vi "Game_Undo_Move.vi"(0 "Context":T1={"Screen"=enum."Settings", "Settings"=[0, 0, 1, 1], "Board"={"Grid"=array15x15[225 elements], "Move History"=[], "Last Move"={"Row"=-1, "Col"=-1, "Stone"=enum."Empty"}}, "Status"=enum."Idle", "Game ID"=0, "Player Stone"=enum."Black", "Hover"={"Row"=-1, "Col"=-1, "Stone"=enum."Empty"}, "Hover Button"=-1, "Win Line"=[], "Score 1"=0, "Score 2"=0, "Draws"=0, "Status Text"="", "Status Color"=0}, 11 "error in":errorcluster) -> (4 "Context out":T1={"Screen"=enum."Settings", "Settings"=[0, 0, 1, 1], "Board"={"Grid"=array15x15[225 elements], "Move History"=[], "Last Move"={"Row"=-1, "Col"=-1, "Stone"=enum."Empty"}}, "Status"=enum."Idle", "Game ID"=0, "Player Stone"=enum."Black", "Hover"={"Row"=-1, "Col"=-1, "Stone"=enum."Empty"}, "Hover Button"=-1, "Win Line"=[], "Score 1"=0, "Score 2"=0, "Draws"=0, "Status Text"="", "Status Color"=0}, 15 "error out":errorcluster)   [LabVIEW 2026]
doc: "무르기 버튼: 2인 플레이는 1수, AI 대전은 플레이어 차례가 되도록 1~2수(AI 흑 첫 수는 유지).\nGame ID를 올려 계산 중이던 AI 결과를 버린다."
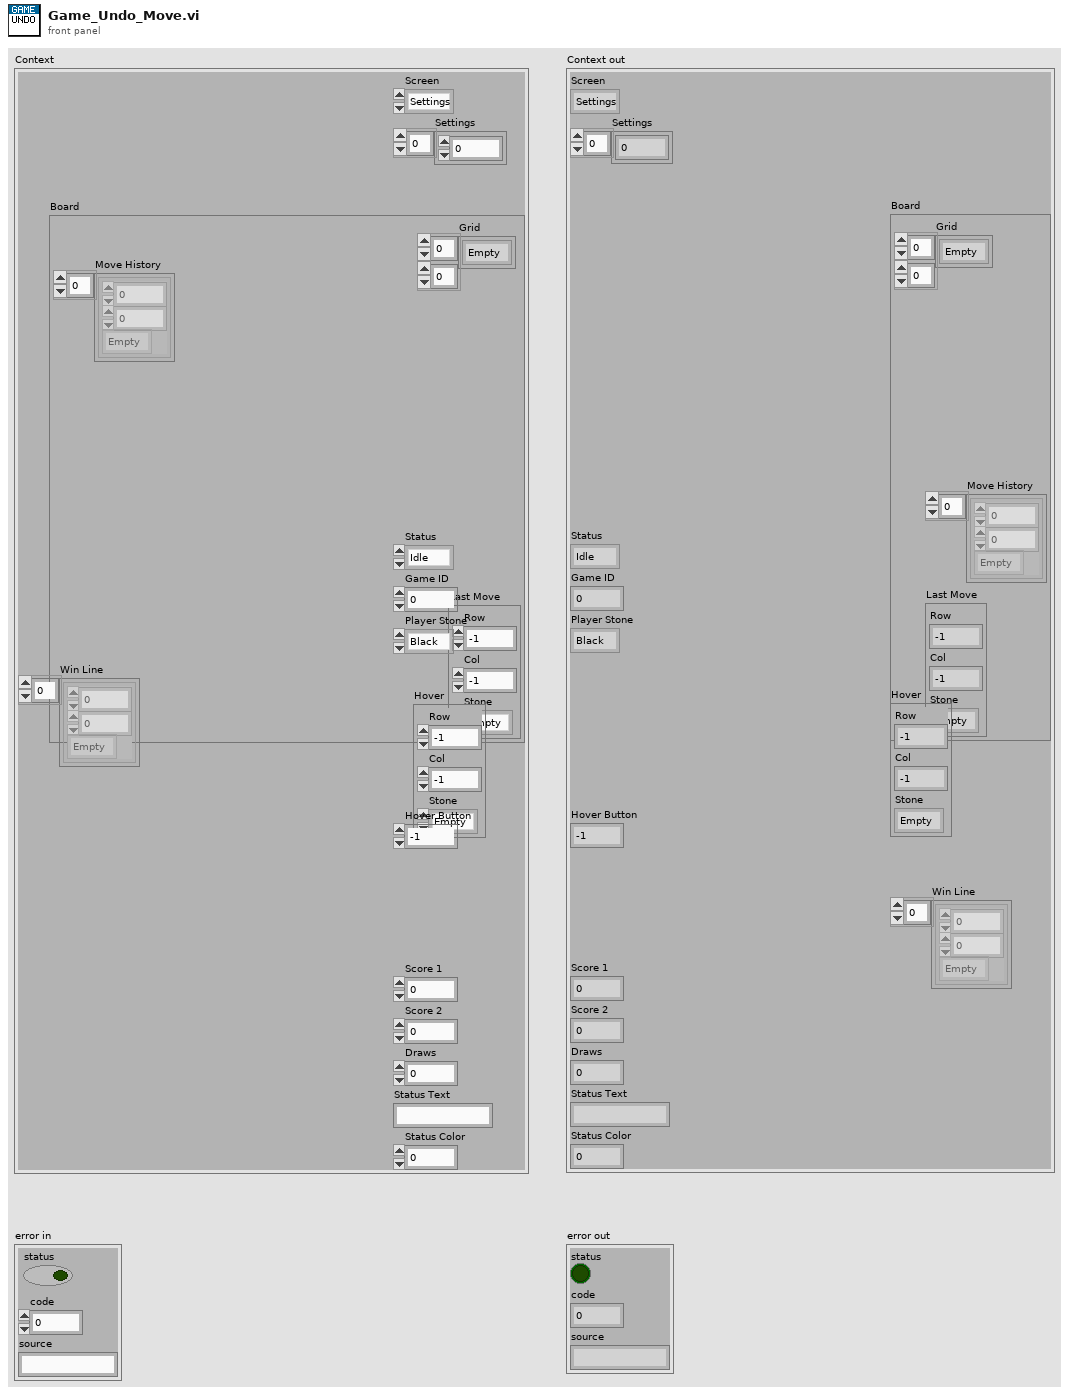
[diagram p1: front panel]
types:
  T1 = cluster{"Screen":enum16{"Settings", "Game"}, "Settings":i32[], "Board":cluster{"Grid":enum8{"Empty", "Black", "White"}[][], "Move History":cluster{"Row":i32, "Col":i32, "Stone":enum8{"Empty", "Black", "White"}}[], "Last Move":cluster{"Row":i32, "Col":i32, "Stone":enum8{"Empty", "Black", "White"}}}, "Status":enum16{"Idle", "Player Turn", "AI Thinking", "Game Over"}, "Game ID":u32, "Player Stone":enum8{"Empty", "Black", "White"}, "Hover":cluster{"Row":i32, "Col":i32, "Stone":enum8{"Empty", "Black", "White"}}, "Hover Button":i32, "Win Line":cluster{"Row":i32, "Col":i32, "Stone":enum8{"Empty", "Black", "White"}}[], "Score 1":i32, "Score 2":i32, "Draws":i32, "Status Text":string, "Status Color":u32}
  T2 = enum16{"Idle", "Player Turn", "AI Thinking", "Game Over"}
  T3 = cluster{"Row":i32, "Col":i32, "Stone":enum8{"Empty", "Black", "White"}}[]
  T4 = cluster{"Grid":enum8{"Empty", "Black", "White"}[][], "Move History":cluster{"Row":i32, "Col":i32, "Stone":enum8{"Empty", "Black", "White"}}[], "Last Move":cluster{"Row":i32, "Col":i32, "Stone":enum8{"Empty", "Black", "White"}}}
  T5 = cluster{"Row":i32, "Col":i32, "Stone":enum8{"Empty", "Black", "White"}}
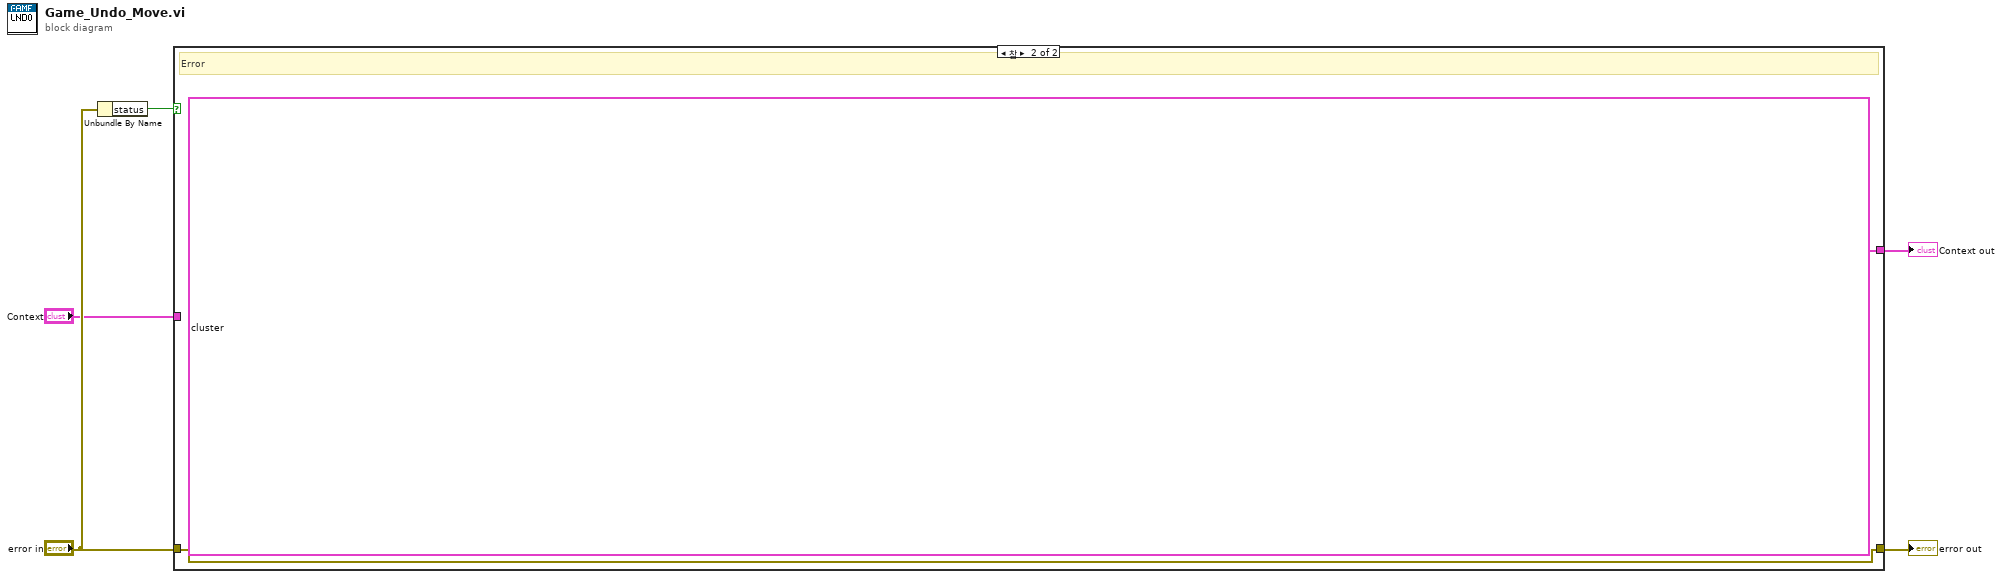
[diagram p0: block diagram]
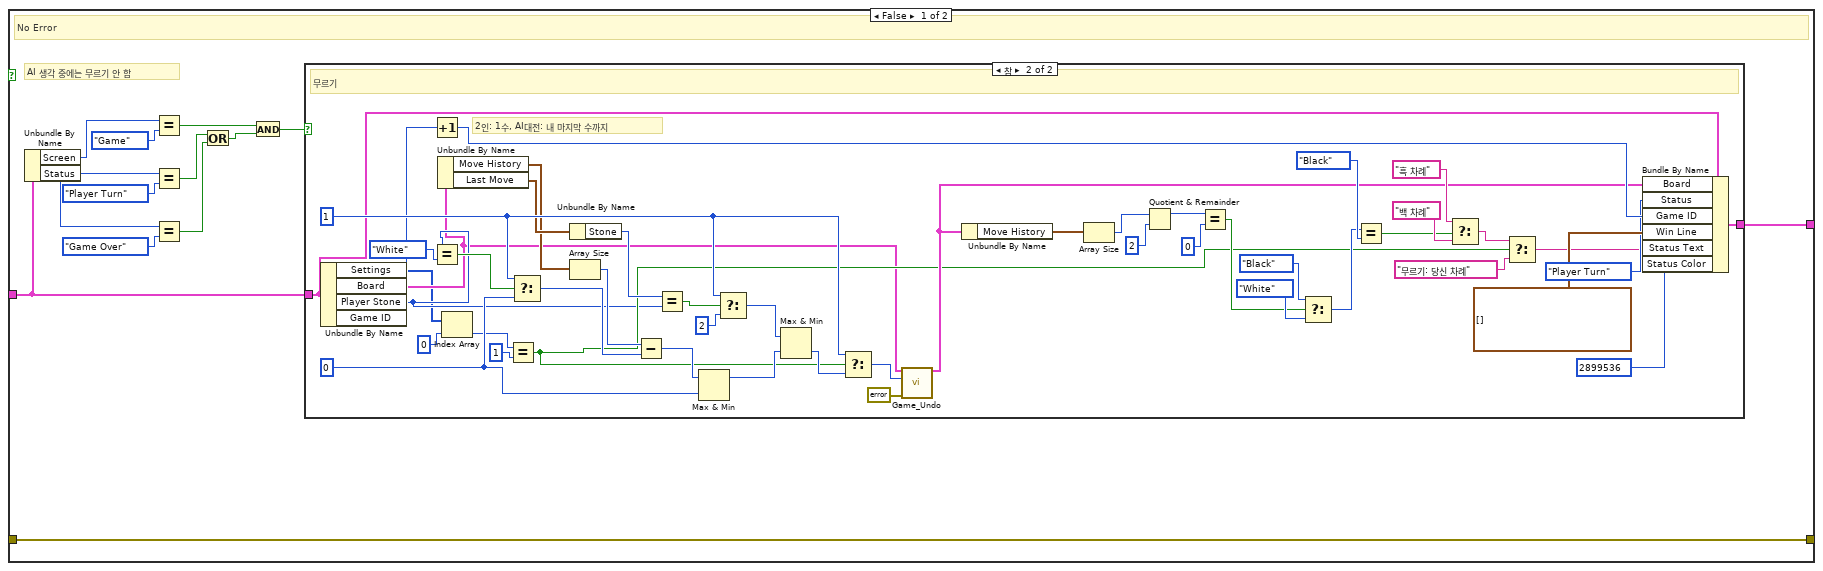
[diagram p2: hidden frame]
diagram:
  n1 = Unbundle By Name("error in") -> ("status"=w3:bool)
  n2 = case shown="참" w3 {
    tunnel: "Context" -> [w6 _]
    tunnel: "error in" -> [w7 w68]
    tunnel: [w7 w68] -> w5
    tunnel: [w18 T1 {"Screen"=enum."Settings", "Settings"=[0, 0, 1, 1], "Board"={"Grid"=array15x15[225 elements], "Move History"=[], "Last Move"={"Row"=-1, "Col"=-1, "Stone"=enum."Empty"}}, "Status"=enum."Idle", "Game ID"=0, "Player Stone"=enum."Black", "Hover"={"Row"=-1, "Col"=-1, "Stone"=enum."Empty"}, "Hover Button"=-1, "Win Line"=[], "Score 1"=0, "Score 2"=0, "Draws"=0, "Status Text"="", "Status Color"=0}] -> w4
    frame False {
      # "AI 생각 중에는 무르기 안 함"
      # "No Error"
      n3 = Unbundle By Name(w6) -> ("Screen"=w8:enum16{"Settings", "Game"}, "Status"=w9:T2)
      n4 = Equal?(x=w8, y=enum16{"Settings", "Game"}."Game") -> (x = y?=w11:bool)
      n5 = Equal?(x=w9, y=T2."Player Turn") -> (x = y?=w13:bool)
      n6 = Equal?(x=w9, y=T2."Game Over") -> (x = y?=w15:bool)
      n7 = Or(x=w13, y=w15) -> (x .or. y?=w16:bool)
      n8 = And(x=w11, y=w16) -> (x .and. y?=w17:bool)
      n9 = case shown="참" w17 {
        tunnel: w6 -> [w19 w20]
        tunnel: [w19 w67] -> w18
        frame False {
          # "무시"
        }
        frame True {
          w35 = 0
          w33 = 1
          # "2인: 1수, AI대전: 내 마지막 수까지"
          # "무르기"
          n10 = Unbundle By Name(w20) -> ("Settings"=w21:i32[], "Board"=w22:T4, "Player Stone"=w23:enum8{"Empty", "Black", "White"}, "Game ID"=w24:u32)
          n11 = Increment(x=w24) -> (x+1=w64:u32)
          n12 = Equal?(x=w23, y=enum8{"Empty", "Black", "White"}."White") -> (x = y?=w39:bool)
          n13 = Unbundle By Name(w22) -> ("Move History"=w29:T3, "Last Move"=w30:T5)
          n14 = Index Array(array=w21, index=0) -> (element=w26:i32)
          n15 = Equal?(x=w26, y=1) -> (x = y?=w28:bool)
          n16 = Select(t=w33, s=w39, f=w35) -> (s? t:f=w40:i32)
          n17 = Unbundle By Name(w30) -> ("Stone"=w32:enum8{"Empty", "Black", "White"})
          n18 = Array Size(array=w29) -> (size(s)=w31:i32)
          n19 = Subtract(x=w31, y=w40) -> (x-y=w41:i32)
          n20 = Equal?(x=w32, y=w23) -> (x = y?=w36:bool)
          n21 = Max & Min(x=w41, y=w35) -> (max(x,y)=w42:i32)  [unwired: 1 out]
          n22 = Select(t=w33, s=w36, f=2) -> (s? t:f=w37:i32)
          n23 = Max & Min(x=w37, y=w42) -> (min(x,y)=w43:i32)  [unwired: 1 out]
          n24 = Select(t=w33, s=w28, f=w43) -> (s? t:f=w44:i32)
          n25 = call "Game_Undo.vi"("Board State"=w22, "Count"=w44, "error in"=errorcluster {"status"=FALSE, "code"=0, "source"=""}) -> ("Board State out"=w46:T4)  [unwired: 10 in, 2 out]
          n26 = Unbundle By Name(w46) -> ("Move History"=w47:T3)
          n27 = Array Size(array=w47) -> (size(s)=w48:i32)
          n28 = Quotient & Remainder(x=w48, y=2) -> (x-y*floor(x/y)=w50:i32)  [unwired: 1 out]
          n29 = Equal?(x=w50, y=0) -> (x = y?=w52:bool)
          n30 = Select(t=enum8{"Empty", "Black", "White"}."Black", s=w52, f=enum8{"Empty", "Black", "White"}."White") -> (s? t:f=w55:enum8{"Empty", "Black", "White"})
          n31 = Equal?(x=w55, y=enum8{"Empty", "Black", "White"}."Black") -> (x = y?=w57:bool)
          n32 = Select(t="흑 차례", s=w57, f="백 차례") -> (s? t:f=w60:string)
          n33 = Select(t=w60, s=w28, f="무르기: 당신 차례") -> (s? t:f=w62:string)
          n34 = Bundle By Name(cluster=w20, "Board"=w46, "Status"=T2."Player Turn", "Game ID"=w64, "Win Line"=T3 [], "Status Text"=w62, "Status Color"=u32 2899536) -> (w67:T1)
        }
      }
    }
    frame True {
      # "Error"
    }
  }
  "Context out" <- w4
  "error out" <- w5
